vi "2_3_VisualAD_Inference(Image)_Multi_MemBanks.vi"() -> ()   [LabVIEW 2020]
uses:
  <vilib>/Ngene/DeepLTK Anomaly Detection Addon/Toolkit/API/Controls/NNPC_Setup.ctl
  <vilib>/Ngene/Deep Learning Toolkit/Toolkit/NN_Data/API/NN_Dims(C,H,W).ctl
  <vilib>/Ngene/Deep Learning Toolkit/Toolkit/NN_Network/Controls/NN_Device.ctl
  <vilib>/Ngene/DeepLTK Anomaly Detection Addon/Toolkit/API/Controls/Feature_Scorer_Params.ctl
  <vilib>/Ngene/DeepLTK Anomaly Detection Addon/Toolkit/API/Controls/Gaussian_Blur.ctl
  <vilib>/Ngene/DeepLTK Anomaly Detection Addon/Toolkit/API/Controls/NN_Paths.ctl
  subVIs/Visualizer/Controls/Display_Options.ctl
  subVIs/Visualizer/Controls/ROI_Display_Options.ctl
  subVIs/Visualizer/Controls/Heatmap_Display_Options.ctl
  subVIs/Visualizer/Controls/ColorMap.ctl
  <vilib>/Ngene/DeepLTK Anomaly Detection Addon/Toolkit/API/Controls/MinMax.ctl
  subVIs/Visualizer/Controls/Report_Images_CFG.ctl
  <vilib>/Ngene/DeepLTK Anomaly Detection Addon/Toolkit/API/NNPC_Predict/NNPC_Predict(Single).vi
  <vilib>/Ngene/DeepLTK Anomaly Detection Addon/Toolkit/DeepLTK_Anomaly_Detection_Addon.lvlib
  <vilib>/Ngene/Deep Learning Toolkit/Toolkit/Deep_Learning_Toolkit_by_Ngene.lvlib
panel:
  out "error out":errorcluster
  in  "MemBank Device":T1=enum."GPU"
  in  "Model Idx":i32 min=0 max=2
  in  "Display_Options":T2={"ROI_Options"={"Color"=16711680, "Width"=3, "Drawing Mode"=enum."Frame"}, "Heatmap_Options"={"ColorMap"=enum."Jet", "Alpha"=0.4, "Heatmap Range"={"Min"=30.0, "Max"=35.0}}, "Report_Images_CFG"={"Original Image"=TRUE, "Ground Truth"=FALSE, "HeatMap"=TRUE, "Mask"=TRUE, "Segmentation"=TRUE}} {"Heatmap_Options"."Heatmap Range"."Min" format="%#_5g"}
  out "dT_Init":dbl=0.946845200000098 format="%#_3ps"
  in  "Paths_to_Individual_Trained_Models":T8[](array[typedef])=[{"CFG"=path "D:/working/Ngene_Trained_Models/NNPC_Cards.cfg", "BIN"=path ""}, {"CFG"=path "D:/working/Ngene_Trained_Models/NNPC_Pill.cfg", "BIN"=path ""}, {"CFG"=path "D:/working/Ngene_Trained_Models/NNPC_PCB.cfg", "BIN"=path ""}]
  out "Image_Thrshld (Eval)":sgl=37.9037
  in  "Image_Thrshld(Custom)":sgl=-1.0 format="%_5g"
  out "dT_Predict(Total)":dbl=0.023180500000307802 format="%#_3ps"
  out "Pixel_Score(Min)":sgl=7.3697577
  out "Pixel_Score(Max)":sgl=39.623528
  out "Image_File_Path":path=path "\\\\ngds\\Data/DNN/AD/Ngene/Engineering_Week/2025_10_02/PCB/Test/bend_cap/bend_cap_10.bmp"
  in  "Feature_Scorer_Params":T9={"Nearest_Neighbors"=1, "Calculate Anomaly Map"=TRUE, "Gaussian_Blur"={"Kernel_Size"=33, "Sigma"=4.0}}
  out "Pixel_Thrshld (Eval)":sgl=42.4708
  in  "Stop":bool
  out "Anomaly?":bool=TRUE
  out "dT_ImRead(Total)":dbl=0.03123639999921579 format="%#_4ps"
  in  "NNPC_Setup":T11={"Input_Dims"={"C"=-1, "H"=-1, "W"=-1}, "mBatch"=1, "Device"=enum."GPU", "GPU Id"=0}
  out "Anomaly Detection Results":T13(plugin-control)
  out "Img_Score":sgl=41.70695
  in  "Image_idx":i32 min=0 max=509
  in  "Ground_Truth_Folders_Paths":path[](array[path])
  in  "Pixel_Thrshld(Custom)":sgl=32.0 format="%_5g"
  in  "Test_Datasets_Folder_Paths":path[](array[path])=[path "\\\\ngds\\Data/DNN/AD/Ngene/Engineering_Week/2025_10_02/Cards/Test", path "\\\\ngds\\Data/DNN/AD/Ngene/Engineering_Week/2025_10_02/Pill/Test", path "\\\\ngds\\Data/DNN/AD/Ngene/Engineering_Week/2025_10_02/PCB/Test"]
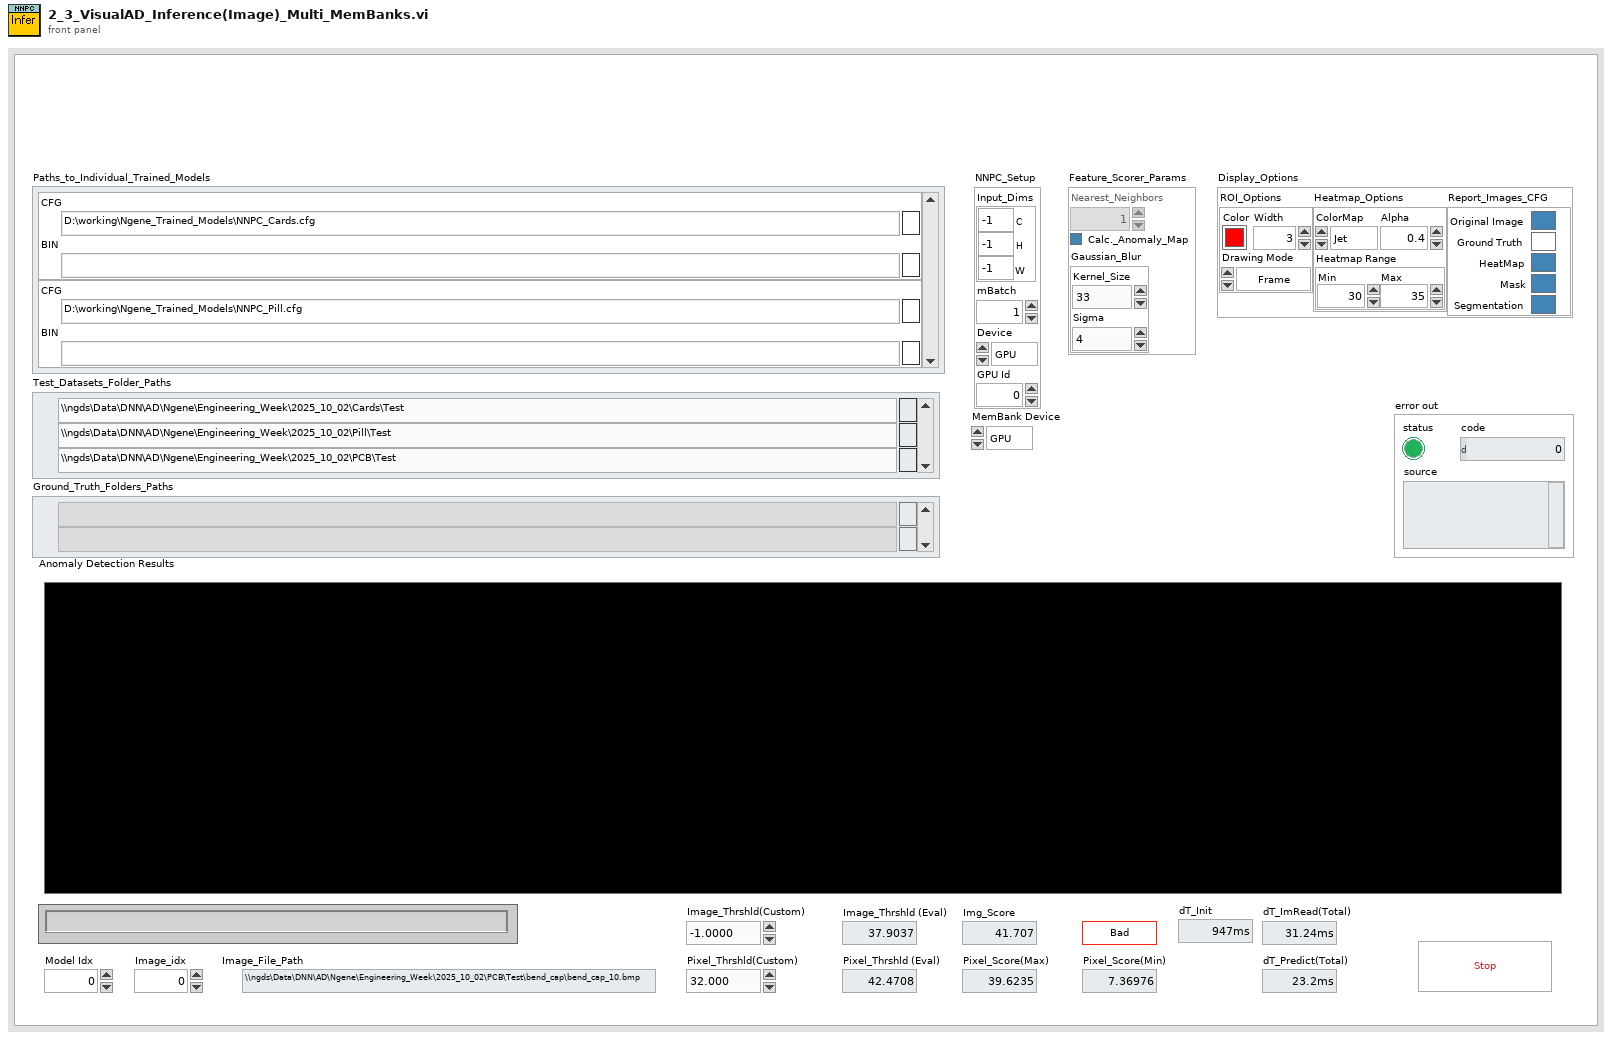
[diagram p1: front panel]
types:
  T1 = typedef "Deep_Learning_Toolkit_by_Ngene.lvlib/NN_Device.ctl" = enum16{"CPU", "GPU"}
  T2 = typedef "Display_Options.ctl" = cluster{"ROI_Options":T3, "Heatmap_Options":T4, "Report_Images_CFG":T7}
  T3 = typedef "ROI_Display_Options.ctl" = cluster{"Color":u32, "Width":u32, "Drawing Mode":enum16{"Frame", "Fill"}}
  T4 = typedef "Heatmap_Display_Options.ctl" = cluster{"ColorMap":T5, "Alpha":sgl, "Heatmap Range":T6}
  T5 = typedef "ColorMap.ctl" = enum16{"Jet", "Perula", "Inferno", "Plasma", "Viridis"}
  T6 = typedef "DeepLTK_Anomaly_Detection_Addon.lvlib/MinMax.ctl" = cluster{"Min":sgl, "Max":sgl}
  T7 = typedef "Report_Images_CFG.ctl" = cluster{"Original Image":bool, "Ground Truth":bool, "HeatMap":bool, "Mask":bool, "Segmentation":bool}
  T8 = typedef "DeepLTK_Anomaly_Detection_Addon.lvlib/NN_Paths.ctl" = cluster{"CFG":path, "BIN":path}
  T9 = typedef "DeepLTK_Anomaly_Detection_Addon.lvlib/Feature_Scorer_Params.ctl" = cluster{"Nearest_Neighbors":i32, "Calculate Anomaly Map":bool, "Gaussian_Blur":T10}
  T10 = typedef "DeepLTK_Anomaly_Detection_Addon.lvlib/Gaussian_Blur.ctl" = cluster{"Kernel_Size":i32, "Sigma":sgl}
  T11 = typedef "DeepLTK_Anomaly_Detection_Addon.lvlib/NNPC_Setup.ctl" = cluster{"Input_Dims":T12, "mBatch":i32, "Device":T1, "GPU Id":i32}
  T12 = typedef "Deep_Learning_Toolkit_by_Ngene.lvlib/NN_Dims(C,H,W).ctl" = cluster{"C":i32, "H":i32, "W":i32}
  T13 = typedef "IMAQ Image.ctl" = refnum<image>
  T14 = typedef "NNPC_MemBank_and_Params.ctl" = cluster{"MemBank_Data":T15, "PreProc_Options":T16, "Evaluation_Results":T20, "MemBank on GPU?":bool}
  T15 = typedef "DeepLTK_Anomaly_Detection_Addon.lvlib/MemBank_and_Norm_Variants.ctl" = cluster{"MemBank":variant, "MemBank Norm":variant}
  T16 = typedef "DeepLTK_Anomaly_Detection_Addon.lvlib/NNPC_PreProcessing_Options.ctl" = cluster{"DS_Name":string, "Input_Dims":T12, "Cropping":T17, "Interpolation Type":u32, "MultiStage_ReSample?":bool, "Dataset_Stats":T18}
  T17 = typedef "DeepLTK_Anomaly_Detection_Addon.lvlib/Crop_CFG.ctl" = cluster{"Left":sgl, "Top":sgl, "Right":sgl, "Bottom":sgl}
  T18 = typedef "DeepLTK_Anomaly_Detection_Addon.lvlib/NNPC_DS_Stats.ctl" = cluster{"means":T19, "stds":T19}
  T19 = typedef "DeepLTK_Anomaly_Detection_Addon.lvlib/Image_Stats_RGB.ctl" = cluster{"R":sgl, "G":sgl, "B":sgl}
  T20 = typedef "DeepLTK_Anomaly_Detection_Addon.lvlib/NNPC_Evaluation_Results.ctl" = cluster{"Threshold(Image)":sgl, "Threshold(Pixel)":sgl, "Pixel_Range":cluster{"Min":sgl, "Max":sgl}}
  T21 = typedef "DeepLTK_Anomaly_Detection_Addon.lvlib/NNPC_Instance.ctl" = cluster{"Name":string, "NN":T22, "MemBank_Data":T15}
  T22 = typedef "Deep_Learning_Toolkit_by_Ngene.lvlib/NN.ctl" = cluster{"Name":string, "No of Layers":i32, "mBatch":i32, "Layers":T23[], "Dimty":T24, "Dims_In":T12, "Dims_Out":T12, "Working_Dir":path, "Train?":bool, "Train_Params":T25, "LR_Update_Policy":T28, "Session Data":T30, "Ground_truth":T31, "NNg_hdls":T32, "NN_Device":T1, "GPU Id":i32, "Labels":string[], "Loss_Type":T33, "Loss_Cfg_Prms":variant, "NNG_WS":T34, "DryRun?":bool}
  T23 = typedef "Deep_Learning_Toolkit_by_Ngene.lvlib/NN_Layer_ref.ctl" = refnum<file>
  T24 = typedef "Deep_Learning_Toolkit_by_Ngene.lvlib/NN_In_Out_Dim-ty.ctl" = enum8{"In1D_Out1D", "In3D_Out1D", "In3D_Out3D", "In3D_OutBBox"}
  T25 = typedef "Deep_Learning_Toolkit_by_Ngene.lvlib/NN_Train_Params.ctl" = cluster{"Optimizer":T26, "Beta_1":sgl, "Beta_2":sgl, "Weight Decay(L1)":sgl, "Weight Decay(L2)":sgl, "Data_Sampling":T27}
  T26 = typedef "Deep_Learning_Toolkit_by_Ngene.lvlib/NN_Train_Optimizer.ctl" = enum16{"SGD", "Adam", "Adagrad", "Adadelta", "RMSProp", "Nesterov"}
  T27 = typedef "Deep_Learning_Toolkit_by_Ngene.lvlib/NN_Train_Data_Sampling.ctl" = enum16{"Random", "Sequential"}
  T28 = typedef "Deep_Learning_Toolkit_by_Ngene.lvlib/NN_LR_Policy_Cfg.ctl" = cluster{"Policy_Type":T29, "LR0":dbl, "k":sgl, "WarmUp_Policy":enum16{"Step", "Ramp"}, "WarmUp_Iter":i32, "WarmUp_Ratio":sgl}
  T29 = typedef "Deep_Learning_Toolkit_by_Ngene.lvlib/NN_LR_Policy_Type.ctl" = enum16{"Manual", "Step", "Exp", "1/t"}
  T30 = typedef "Deep_Learning_Toolkit_by_Ngene.lvlib/NN_Train_Session_Data.ctl" = cluster{"Epochs":sgl, "Tot_Iter":i32, "LR":sgl, "LR_iter":i32}
  T31 = typedef "Deep_Learning_Toolkit_by_Ngene.lvlib/NN_Ground_truth.ctl" = cluster{"Y":variant}
  T32 = typedef "Deep_Learning_Toolkit_by_Ngene.lvlib/nng_cuda_handles.ctl" = cluster{"cudnn":u64, "cublas":u64, "stream":u64, "curand":u64}
  T33 = typedef "Deep_Learning_Toolkit_by_Ngene.lvlib/NN_Loss_Type.ctl" = enum16{"None", "MSE", "CrossEntropy", "YOLO_v2", "YOLO_v4"}
  T34 = typedef "Deep_Learning_Toolkit_by_Ngene.lvlib/NNG_WS.ctl" = cluster{"NNG_WS_Mem":T35, "Max_WS_Size":i64}
  T35 = typedef "Deep_Learning_Toolkit_by_Ngene.lvlib/NNg_WS_Mem_DVR.ctl" = refnum<data-value>
  T36 = typedef "Anomaly_Detection_Results_Imgs.ctl" = cluster{"Image":T13, "Ground Truth":T13, "Predicted Heat Map":T13, "Predicted Mask":T13, "Segmentation":T13}
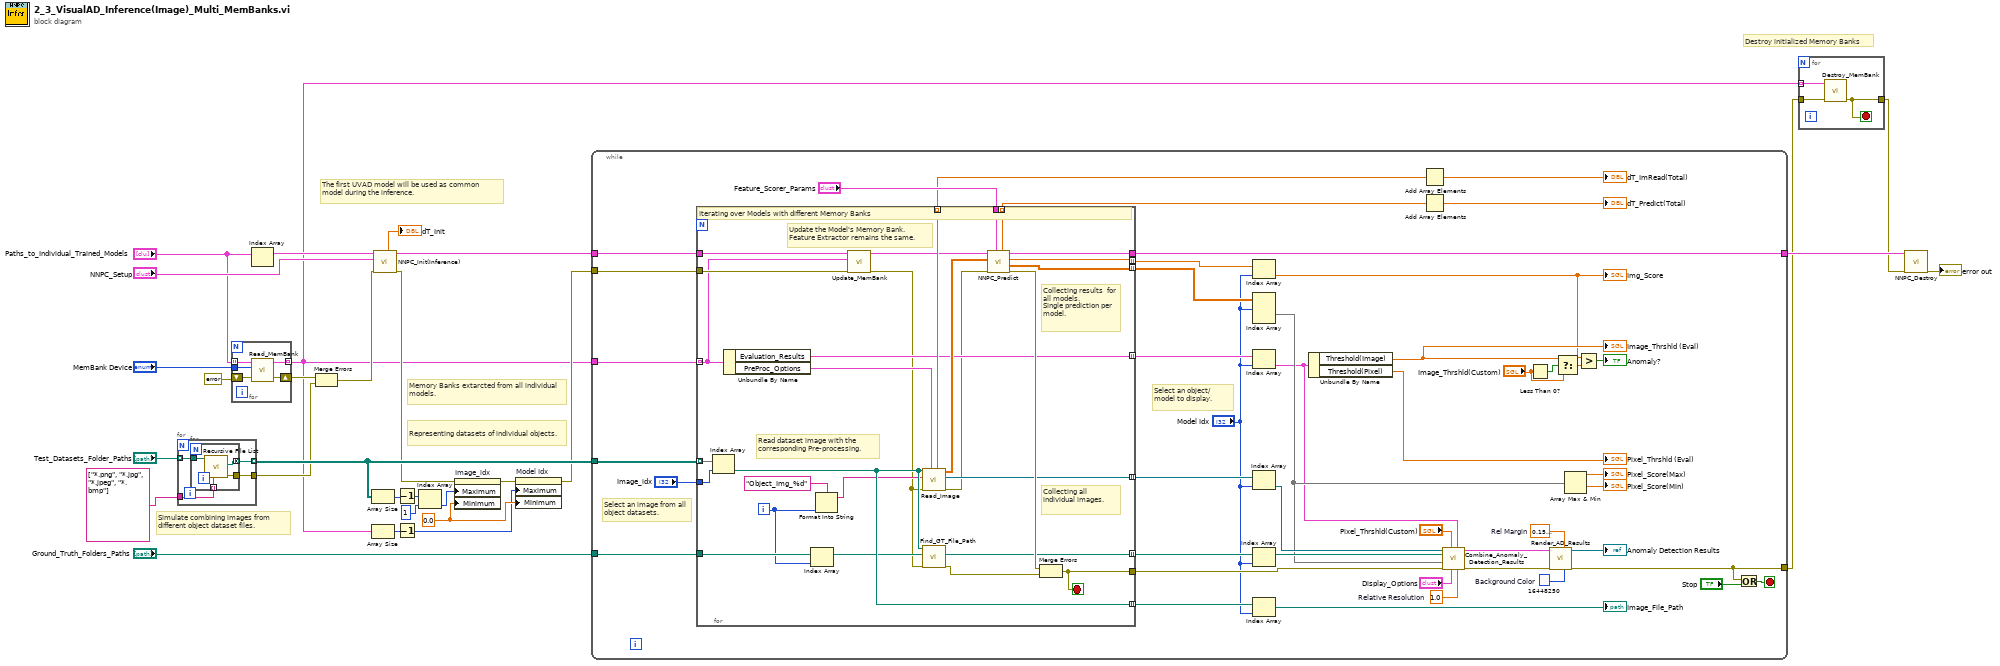
[diagram p0: block diagram]
diagram:
  w16 = 0.0 ("Data Entry Limits:Minimum")
  # "Destroy initialized Memory Banks"
  # "Memory Banks extarcted from all individual models."
  # "Representing datasets of individual objects."
  # "The first UVAD model will be used as common model during the inference."
  # "Simulate combining images from different object dataset files."
  n1 = for {
    tunnel: "Test_Datasets_Folder_Paths" -> [w32] mode=indexing
    tunnel: [w30] -> w23 mode=indexing
    tunnel: [w33] -> w22
    tunnel: string[] ["*.png", "*.jpg", "*.jpeg", "*.bmp"] ("pattern") -> [w31]
    n2 = for {
      tunnel: [w37] -> w33
      tunnel: w32 -> [w36]
      tunnel: w31 -> [w35] mode=indexing
      tunnel: [w34] -> w30 mode=concatenating
      n3 = call <vilib>:"Recursive File List.vi"("pattern"=w35, "Folder Path"=w36) -> ("error out"=w37:errorcluster, "All Files in Dir"=w34:path[])  [unwired: 5 in, 3 out]
    }
  }
  n4 = for {
    tunnel: "Paths_to_Individual_Trained_Models" -> [w42] mode=indexing
    tunnel: [w41] -> w5 mode=indexing
    shift-right: [w40] -> w13
    shift-left: errorcluster {"status"=FALSE, "code"=0, "source"=""} ("error out") -> [w39]
    tunnel: "MemBank Device" -> [w38]
    n5 = call "Read_MemBank.vi"("error in"=w39, "Device"=w38, "NNPC_Paths"=w42) -> ("error out"=w40:errorcluster, "NNPC_MemBank_and_Params"=w41:T14)  [unwired: 7 in]
  }
  n6 = Index Array(array="Paths_to_Individual_Trained_Models") -> (element=w6:T8)  [unwired: 1 in]
  n7 = Merge Errors(w13, w22) -> (w12:errorcluster)
  n8 = Array Size(array=w23) -> (size(s)=w27:i32[])
  n9 = Array Size(array=w5) -> (size(s)=w15:i32)
  n10 = call <vilib>:"NNPC_Init(Inference).vi"("error in"=w12, "NNPC_Setup"="NNPC_Setup", "NNPC_Paths"=w6) -> ("error out"=w11:errorcluster, "NNPC_out"=w21:T21, "dT_Init_Inference"=→"dT_Init":dbl)  [unwired: 4 in, 2 out]
  n11 = Decrement(x=w27) -> (x-1=w28:i32[])
  n12 = Decrement(x=w15) -> (x-1=w14:i32)
  n13 = Index Array(array=w28, index=1) -> (element=w26:i32)
  n14 = property on="Image_idx" class="DigNum (strict)"(error in=w11, "Maximum"=w26, "Minimum"=w16) -> (error out=w18:errorcluster)  [unwired: 1 in, 1 out]
  n15 = property on="Model Idx" class="DigNum (strict)"(error in=w18, "Maximum"=w14, "Minimum"=w16) -> (error out=w17:errorcluster)  [unwired: 1 in, 1 out]
  n16 = while {
    tunnel: w23 -> [w87]
    tunnel: w21 -> [w57]
    tunnel: [w71] -> w29
    tunnel: w17 -> [w67]
    tunnel: [w68] -> w3
    tunnel: "Ground_Truth_Folders_Paths" -> [w78]
    tunnel: w5 -> [w56]
    stop <- w69 stop-if-true
    w58 = sgl 1.0  # Relative Resolution
    w60 = u32 16448250  # Background Color
    w61 = sgl 0.15  # Rel Margin
    # "Select an image from all object datasets."
    # "Select an object/model to display."
    n17 = for {
      tunnel: w87 -> [w115] mode=indexing
      tunnel: [w113] -> w45 mode=indexing
      tunnel: [w110] -> w75 mode=indexing
      tunnel: [w109] -> w74 mode=indexing
      tunnel: "Feature_Scorer_Params" -> [w108]
      tunnel: [w105] -> w65 mode=indexing
      tunnel: [w104] -> w62 mode=indexing
      tunnel: w56 -> [w88] mode=indexing
      tunnel: "Image_idx" -> [w99]
      tunnel: w78 -> [w111]
      tunnel: [w112] -> w79 mode=indexing
      tunnel: [w98] -> w50 mode=indexing
      tunnel: [w97] -> w48 mode=indexing
      tunnel: w67 -> [w89]
      tunnel: [w96] -> w66
      tunnel: w57 -> [w103]
      tunnel: [w107] -> w71
      i -> [w92]
      stop <- w96 stop-if-true
      # "Collecting all individual images."
      # "Collecting results  for all models.\nSingle prediction per model."
      # "Read dataset image with the corresponding Pre-processing."
      # "Update the Model's Memory Bank.\nFeature Extractor remains the same."
      # "Iterating over Models with different Memory Banks"
      n18 = Index Array(array=w115, index=w99) -> (element=w97:path)
      n19 = Unbundle By Name(w88) -> ("Evaluation_Results"=w98:T20, "PreProc_Options"=w100:T16)
      n20 = Index Array(array=w111, index=w92) -> (element=w93:path)
      n21 = Format Into String(format string="Object_Img_%d", w92) -> (resulting string=w95:string)  [unwired: 2 in, 1 out]
      n22 = call "Update_MemBank.vi"("error in"=w89, "NNPC_MemBank_and_Params"=w88, "NNPC_out in"=w103) -> ("error out"=w90:errorcluster, "NNPC_out out"=w102:T21)  [unwired: 7 in]
      n23 = call "Read_Image.vi"("PreProcessing_Options"=w100, "error in"=w90, "IMAQ Name"=w95, "Img Path"=w97) -> ("error out"=w91:errorcluster, 2:"Image Out (Preproc)"=w104:T13, 3:"Image Out (Preproc)"=w101:sgl[][][], "dT_Img_Read"=w113:dbl)  [unwired: 2 in, 2 out]
      n24 = call "Find_GT_File_Path.vi"("error in"=w90, "GT Mask Folder Path"=w93, "Image File Path"=w97) -> ("error out"=w106:errorcluster, "GT File Path"=w112:path)  [unwired: 5 in, 2 out]
      n25 = call-poly <vilib>:"NNPC_Predict.vi"("Feature_Scorer_Params"=w108, "error in"=w91, "Image_in"=w101, "NNPC_in"=w102) -> ("error out"=w114:errorcluster, "Anomaly_Map"=w110:sgl[][], "Pred_Score"=w109:sgl, "NNPC_out"=w107:T21, "dT_Predict"=w105:dbl)  [unwired: 2 in, 1 out]
      n26 = Merge Errors(w114, w106) -> (w96:errorcluster)
    }
    n27 = Index Array(array=w74, index="Model Idx") -> (element=w51:sgl)
    "Img_Score" <- w51
    n28 = Index Array(array=w75, index (dim 0)="Model Idx") -> (element=w52:sgl[][])  [unwired: 2 in]
    n29 = Index Array(array=w50, index="Model Idx") -> (element=w49:T20)
    n30 = Index Array(array=w62, index="Model Idx") -> (element=w53:T13)
    n31 = Index Array(array=w79, index="Model Idx") -> (element=w54:path)
    n32 = Index Array(array=w48, index="Model Idx") -> (element=→"Image_File_Path":path)
    n33 = Unbundle By Name(w49) -> ("Threshold(Image)"=w64:sgl, "Threshold(Pixel)"=→"Pixel_Thrshld (Eval)":sgl)
    "Image_Thrshld (Eval)" <- w64
    n34 = Add Array Elements(numeric array=w45) -> (sum=→"dT_ImRead(Total)":dbl)
    n35 = Add Array Elements(numeric array=w65) -> (sum=→"dT_Predict(Total)":dbl)
    n36 = call "Combine_Anomaly_Detection_Results.vi"("Relative Resolution"=w58, "Evaluation_Results"=w49, "Display_Options"="Display_Options", "Pixel Anomaly Thrshld"="Pixel_Thrshld(Custom)", "error in"=w66, "Anomaly Map"=w52, "Gt File Path"=w54, "Orig Image In"=w53) -> ("error out"=w86:errorcluster, "Anomaly Detection Results"=w85:T36)  [unwired: 1 in, 1 out]
    n37 = Less Than 0?(x="Image_Thrshld(Custom)") -> (x < 0?=w82:bool)
    n38 = call "Render_AD_Results.vi"("Background Color"=w60, "Rel._Margin"=w61, "error in"=w86, "Anomaly Detection Rresults"=w85) -> ("error out"=w68:errorcluster, "Anomaly Detection Result"=→"Anomaly Detection Results":T13)  [unwired: 6 in]
    n39 = Select(t=w64, s=w82, f="Image_Thrshld(Custom)") -> (s? t:f=w80:sgl)
    n40 = Array Max & Min(array=w52) -> (max value=→"Pixel_Score(Max)":sgl, min value=→"Pixel_Score(Min)":sgl)  [unwired: 2 out]
    n41 = Greater?(x=w51, y=w80) -> (0:→"Anomaly?":bool)
    n42 = Or(x=w68, y="Stop") -> (x .or. y?=w69:bool)
  }
  n43 = for {
    tunnel: w5 -> [w118] mode=indexing
    tunnel: w3 -> [w117]
    tunnel: [w116] -> w2
    stop <- w116 stop-if-true
    n44 = call "Destroy_MemBank.vi"("error in"=w117, "NNPC_MemBank_and_Params"=w118) -> ("error out"=w116:errorcluster)  [unwired: 9 in]
  }
  n45 = call <vilib>:"NNPC_Destroy.vi"("error in"=w2, "NNPC_in"=w29) -> ("error out"=→"error out":errorcluster)  [unwired: 9 in]
